vi "gainConvertPL1 (SubVI).vi"(11 "Gain":sgl) -> (3 "DAC":dbl)   [LabVIEW 2017]
panel:
  out "error out":errorcluster
  in  "error in (no error)":errorcluster
  out "FPGainOfsetPL1":sgl
  out "FPGainSlopePL1":sgl
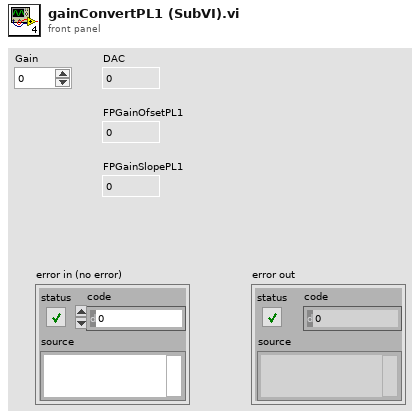
[diagram p1: front panel]
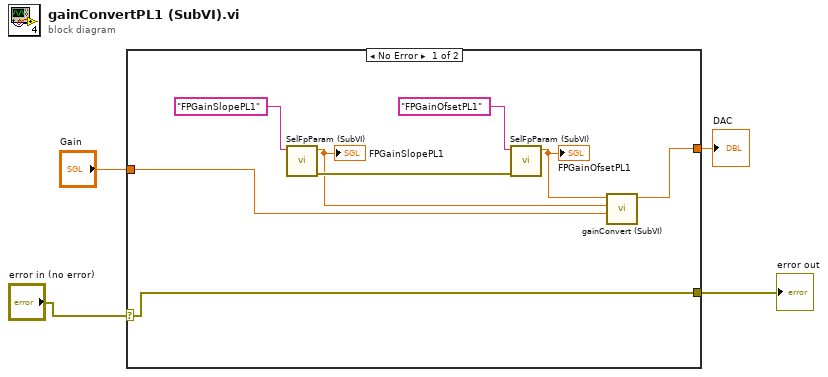
[diagram p0: block diagram]
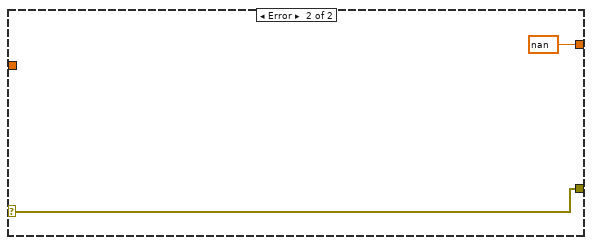
[diagram p2: hidden frame]
diagram:
  n1 = case shown="No Error" "error in (no error)" {
    selector: "error in (no error)" -> [w5 w14]
    tunnel: [w11 nan ("DAC")] -> w4
    tunnel: "Gain" -> [w8 _]
    tunnel: [w5 w14] -> w1
    frame No Error {
      n2 = call "SelFpParam (SubVI).vi"("String"="FPGainSlopePL1") -> ("error out"=w12:errorcluster, "float number"=w10:sgl)  [unwired: 9 in]
      "FPGainSlopePL1" <- w10
      n3 = call "SelFpParam (SubVI).vi"("error in"=w12, "String"="FPGainOfsetPL1") -> ("float number"=w9:sgl)  [unwired: 8 in, 1 out]
      "FPGainOfsetPL1" <- w9
      n4 = call "gainConvert (SubVI).vi"("Gain"=w8, "float number"=w10, "float number 2"=w9) -> ("DAC"=w11:dbl)  [unwired: 8 in]
    }
    frame Error {
    }
  }
  "DAC" <- w4
  "error out" <- w1
